vi "RemoteVI Read Request Head.vi"(0 "connection":u32, 5 "head in":string) -> (4 "head out":string, 6 "complete?":bool, 8 "gone?":bool)   [LabVIEW 2020, in "RemoteVI.lvlib"]
doc: "Reads whatever bytes of an HTTP request head are waiting on a pending connection WITHOUT waiting: TCP Read in immediate mode with timeout 0 (4 KiB at most), appended to head in. complete? is TRUE once the head contains the blank line (CR LF CR LF) or is longer than 16 KiB (RemoteVI Handle Connection.vi then closes it quietly). gone? is TRUE when the read reported any error other than 56 (timeout - nothing waiting), i.e. the peer closed or reset the connection. Called by RemoteVI Serve Pending Connection.vi once per server loop iteration, so a connection that sends nothing never blocks the loop. connection is the TCP connection refnum type-cast to U32."
uses:
  RemoteVI.lvlib
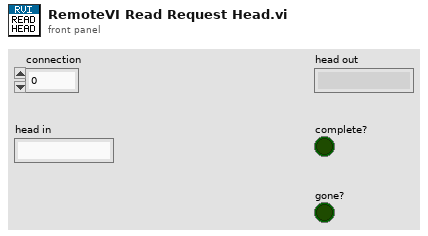
[diagram p1: front panel]
types:
  T1 = enum16{"standard", "buffered", "CRLF", "immediate"}
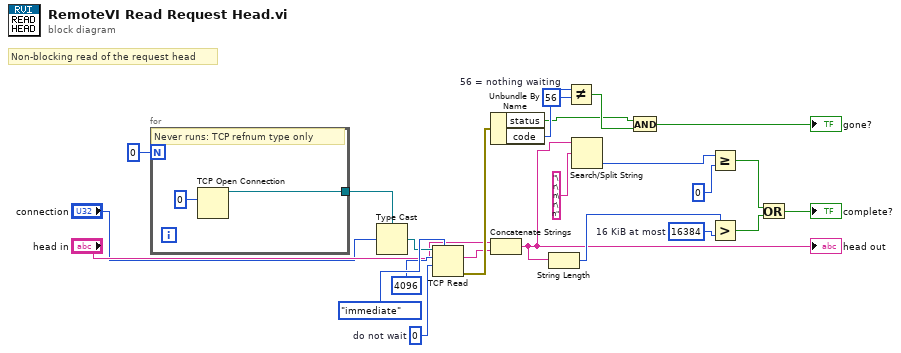
[diagram p0: block diagram]
diagram:
  w22 = 56  # 56 = nothing waiting
  w17 = 16384  # 16 KiB at most
  w7 = 0  # do not wait
  # "Non-blocking read of the request head"
  n1 = for {
    N: 0 -> [_]
    tunnel: [w26] -> w4
    # "Never runs: TCP refnum type only"
    n2 = TCP Open Connection(remote port or service name=u16 0) -> (connection ID=w26:refnum<k5>)  [unwired: 4 in, 1 out]
  }
  n3 = Type Cast(type=w4, x="connection") -> (*(type *) &x=w5:refnum<k5>)
  n4 = TCP Read(connection ID=w5, bytes to read=4096, 7:T1."immediate", 9:w7) -> (data out=w9:string, error out=w10:errorcluster)  [unwired: 1 in, 1 out]
  n5 = Unbundle By Name(w10) -> ("status"=w20:bool, "code"=w21:i32)
  n6 = Concatenate Strings("head in", w9) -> (w11:string)
  "head out" <- w11
  n7 = String Length(string=w11) -> (length=w16:i32)
  n8 = Not Equal?(x=w21, y=w22) -> (x != y?=w23:bool)
  n9 = Search/Split String(string=w11, search string/char (-)="\r\n\r\n") -> (offset of match=w13:i32)  [unwired: 1 in, 2 out]
  n10 = And(x=w20, y=w23) -> (x .and. y?=→"gone?":bool)
  n11 = Greater Or Equal?(x=w13, y=0) -> (x >= y?=w15:bool)
  n12 = Greater?(x=w16, y=w17) -> (0:w18:bool)
  n13 = Or(x=w15, y=w18) -> (x .or. y?=→"complete?":bool)
